vi "RT_Close.vi"(8 "error in (no error)":errorcluster={"status"=FALSE, "code"=0, "source"="\"\""}, 10 "fault status":string, 11 "Hardware handles":string) -> (0 "error out":errorcluster={"status"=FALSE, "code"=0, "source"="\"\""}, 2 "status ok":bool, 3 "Shutdown status":string)   [LabVIEW 2026]
doc: "INTENT: Release RT runtime resources after protective state. LOGIC: Verify safe/protective state, stop control services in approved order and close drivers."
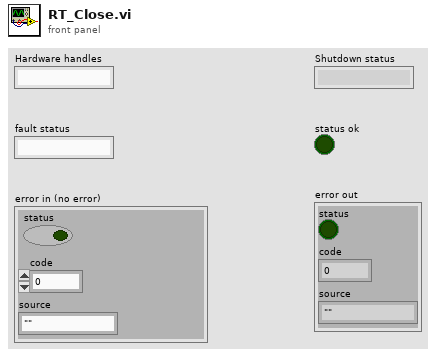
[diagram p1: front panel]
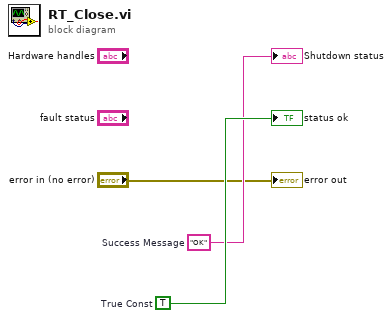
[diagram p0: block diagram]
diagram:
  w3 = TRUE  # True Const
  w2 = "OK"  # Success Message
  "Shutdown status" <- w2
  "status ok" <- w3
  "error out" <- "error in (no error)"
